vi "Remove Session (byClientID).vi"(8 "error in (no error)":errorcluster, 10 "Client ID":string, 11 "MQTT Server":refnum<class "Server.lvclass">) -> (0 "error out":errorcluster, 1 "removed":bool, 2 "Client ID dup":string, 3 "MQTT Server":refnum<class "Server.lvclass">, 5 "SessionMailbox":refnum<queue>)   [LabVIEW 2013, in "MQTT Server.lvlib" / "Server.lvclass"]
uses:
  Server.lvclass
  <vilib>/LabVIEW Open Source Project/MQTT Connection/MQTT_Base/Base Class/Response -- cluster.ctl
  <vilib>/LabVIEW Open Source Project/MQTT Control Packets/Control Packets/ControlPacket/ControlPacket.lvclass
  Server.lvclass/Server.ctl
  <vilib>/LabVIEW Open Source Project/MQTT Connection/MQTT_Base/Base Class/MQTT_Base.lvclass
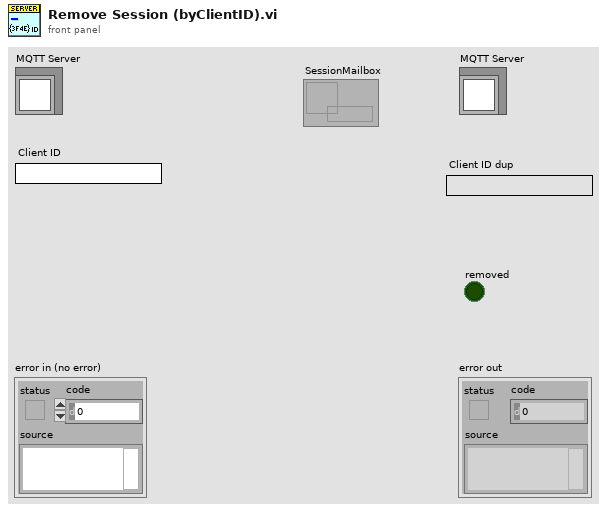
[diagram p1: front panel]
types:
  T1 = typedef "MQTT Server.lvlib/Server.lvclass/SessionRef -- cluster.ctl" = cluster{"ClientID":string, "SessionMailbox":refnum<queue>}
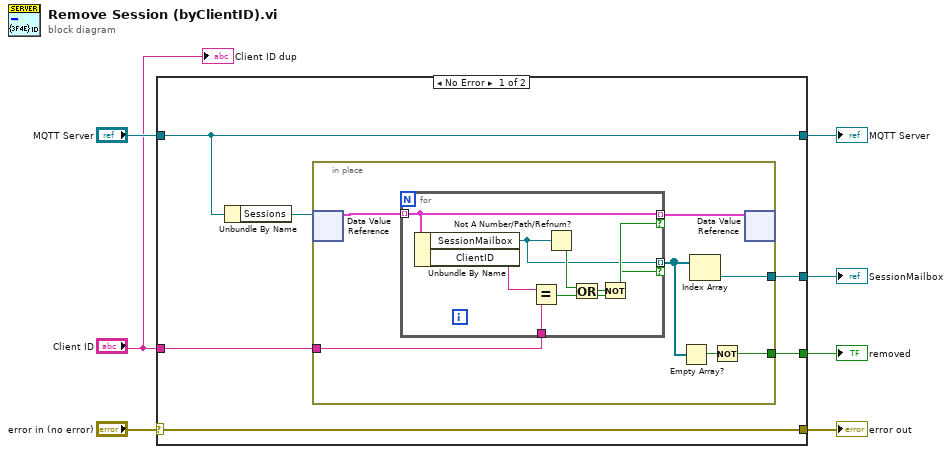
[diagram p0: block diagram]
diagram:
  n1 = case shown="No Error" "error in (no error)" {
    selector: "error in (no error)" -> [w10 w30]
    tunnel: [w10 w30] -> w6
    tunnel: [w12 w29] -> w4
    tunnel: "MQTT Server" -> [w12 w29]
    tunnel: "Client ID" -> [w11 _]
    tunnel: [w9 _] -> w2
    tunnel: [w8 _] -> w1
    frame No Error {
      n2 = Unbundle By Name(w12) -> ("Sessions"=w13:refnum<data-value>)
      n3 = in-place {
        in-place-border: w11 -> [w20]
        in-place-border: [w17] -> w9
        in-place-border: [w16] -> w8
        n4 = in-place-dvr #1(w13) -> (w19:T1[])  [unwired: 1 out]
        n5 = for {
          tunnel: w19 -> [w26] mode=indexing
          tunnel: w20 -> [w27]
          tunnel: [w26] -> w18 mode=indexing if=w23
          tunnel: [w22] -> w14 mode=indexing if=w21
          n6 = Unbundle By Name(w26) -> ("SessionMailbox"=w22:refnum<queue>, "ClientID"=w28:string)
          n7 = Equal?(x=w28, y=w27) -> (x = y?=w21:bool)
          n8 = Not A Number/Path/Refnum?(number/path/refnum=w22) -> (NaN/Path/Refnum?=w25:bool)
          n9 = Or(x=w25, y=w21) -> (x .or. y?=w24:bool)
          n10 = Not(x=w24) -> (.not. x?=w23:bool)
        }
        n11 = Empty Array?(array=w14) -> (empty?=w15:bool)
        n12 = Index Array(array=w14) -> (element=w17:refnum<queue>)  [unwired: 1 in]
        n13 = Not(x=w15) -> (.not. x?=w16:bool)
        n14 = in-place-dvr #1(w18) -> ()  [unwired: 2 out]
      }
    }
    frame Error {
    }
  }
  "error out" <- w6
  "MQTT Server" <- w4
  "SessionMailbox" <- w2
  "removed" <- w1
  "Client ID dup" <- "Client ID"
